vi "VIH HelpGen - HTML - Extract Template Codes - VI Help.vi"(11 "HTML in":string) -> (0 "ProductInfo Template":string, 2 "Table Templates":T1, 3 "HTML out":string)   [LabVIEW 2014]
doc: "::: VI Helpeks :::\nCopyright (c) 2000-2026 Konstantin Shifershteyn. All rights reserved."
uses:
  _VIH HelpGen.llb/VIH HelpGen Typedef - Table Templates Cluster - VI Help.ctl
panel:
  # "VI Helpeks\nCopyright (c) 2012-2026 Konstantin Shifershteyn"
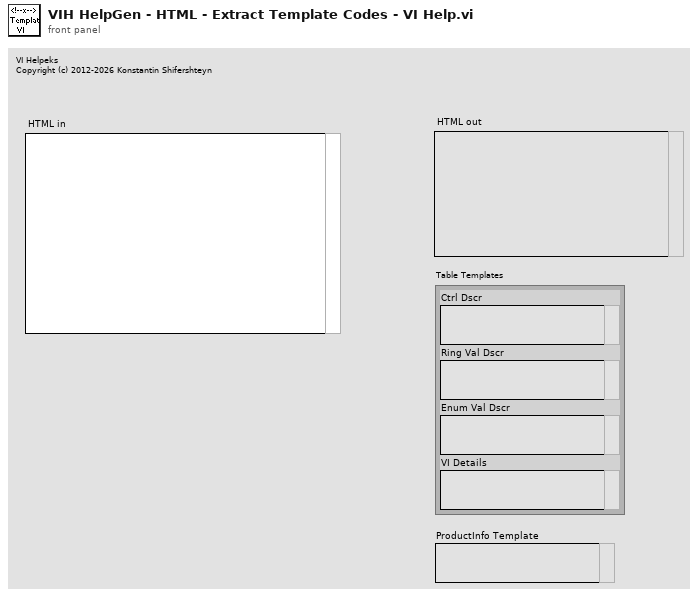
[diagram p1: front panel]
types:
  T1 = typedef "VIH HelpGen Typedef - Table Templates Cluster - VI Help.ctl" = cluster{"Ctrl Dscr":string, "Ring Val Dscr":string, "Enum Val Dscr":string, "VI Details":string}
  T2 = cluster{"String":string, "String":string, "String":string, "String":string}
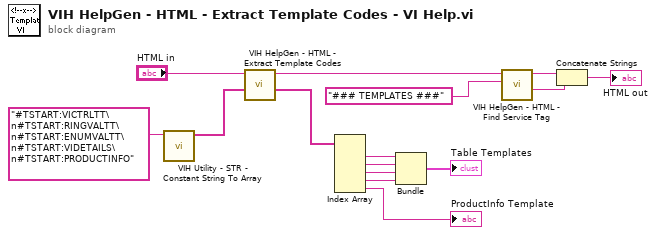
[diagram p0: block diagram]
diagram:
  n1 = call "VIH Utility - STR - Constant String To Array.vi"("String in"="#TSTART:VICTRLTT\n#TSTART:RINGVALTT\n#TSTART:ENUMVALTT\n#TSTART:VIDETAILS\n#TSTART:PRODUCTINFO") -> ("Array out"=w9:string[])  [unwired: 10 in]
  n2 = call "VIH HelpGen - HTML - Extract Template Codes.vi"("Tag names"=w9, "HTML in"="HTML in") -> ("Templates"=w8:string[], "HTML out"=w3:string)  [unwired: 8 in]
  n3 = Index Array(array=w8) -> (element #1=w14:string, element #2=w13:string, element #3=w12:string, element #4=w7:string, element #5=→"ProductInfo Template":string)  [unwired: 5 in]
  n4 = Bundle("String"=w14, "String"=w13, "String"=w12, "String"=w7) -> (→"Table Templates":T2)  [unwired: 1 in]
  n5 = call "VIH HelpGen - HTML - Find Service Tag.vi"("Tag name"="### TEMPLATES ###", "HTML in"=w3) -> ("After"=w6:string, "Before"=w5:string)  [unwired: 6 in, 2 out]
  n6 = Concatenate Strings(w5, w6) -> (→"HTML out":string)
